vi "CreateMethodTree.vi"(6 "DisabledMethodsNames":T1(array[cluster]), 8 "error in (no error)":errorcluster, 9 "StartSelectedMethodsPerInterfaces":T1(array[cluster]), 10 "InterfacePath":T2[](array[typedef]), 11 "TreeControlRef":refnum<vi>) -> (0 "error out":errorcluster, 1 "InterfacesTag":string[](array[string]), 2 "MethodsTagPerInterfaces":cluster{"Array":string[]}[](array[cluster]), 3 "MethodsSelectedPerInterface":cluster{"Array":bool[]}[](array[cluster]), 4 "MethodsDisabledPerInterface":cluster{"Array":bool[]}[](array[cluster]))   [LabVIEW 2020, in "InterfaceLibrary.lvlib"]
uses:
  InterfaceLibrary.lvlib
  InterfaceInfo.ctl
  LvClass_class/GDSLvClass_ClassMethodInfo.ctl
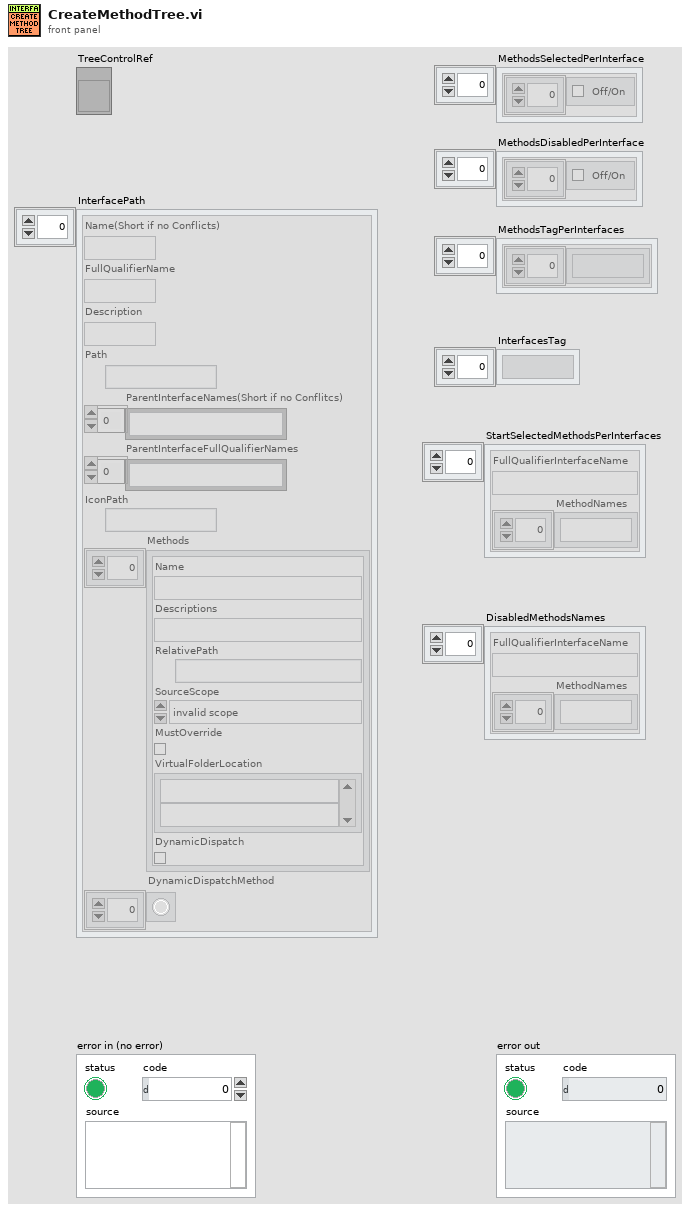
[diagram p1: front panel]
types:
  T1 = cluster{"FullQualifierInterfaceName":string, "MethodNames":string[]}[]
  T2 = typedef "InterfaceLibrary.lvlib/InterfaceInfo.ctl" = cluster{"Name(Short if no Conflicts)":string, "FullQualifierName":string, "Description":string, "Path":path, "ParentInterfaceNames(Short if no Conflitcs)":string[], "ParentInterfaceFullQualifierNames":string[], "IconPath":path, "Methods":T3[], "DynamicDispatchMethod":bool[]}
  T3 = typedef "GDSLvClass_ClassMethodInfo.ctl" = cluster{"Name":string, "Descriptions":string, "RelativePath":path, "SourceScope":enum32{"invalid scope", "public", "private", "protected", "community"}, "MustOverride":bool, "VirtualFolderLocation":string[], "DynamicDispatch":bool}
  T4 = cluster{"FullQualifierInterfaceName":string, "MethodNames":string[]}
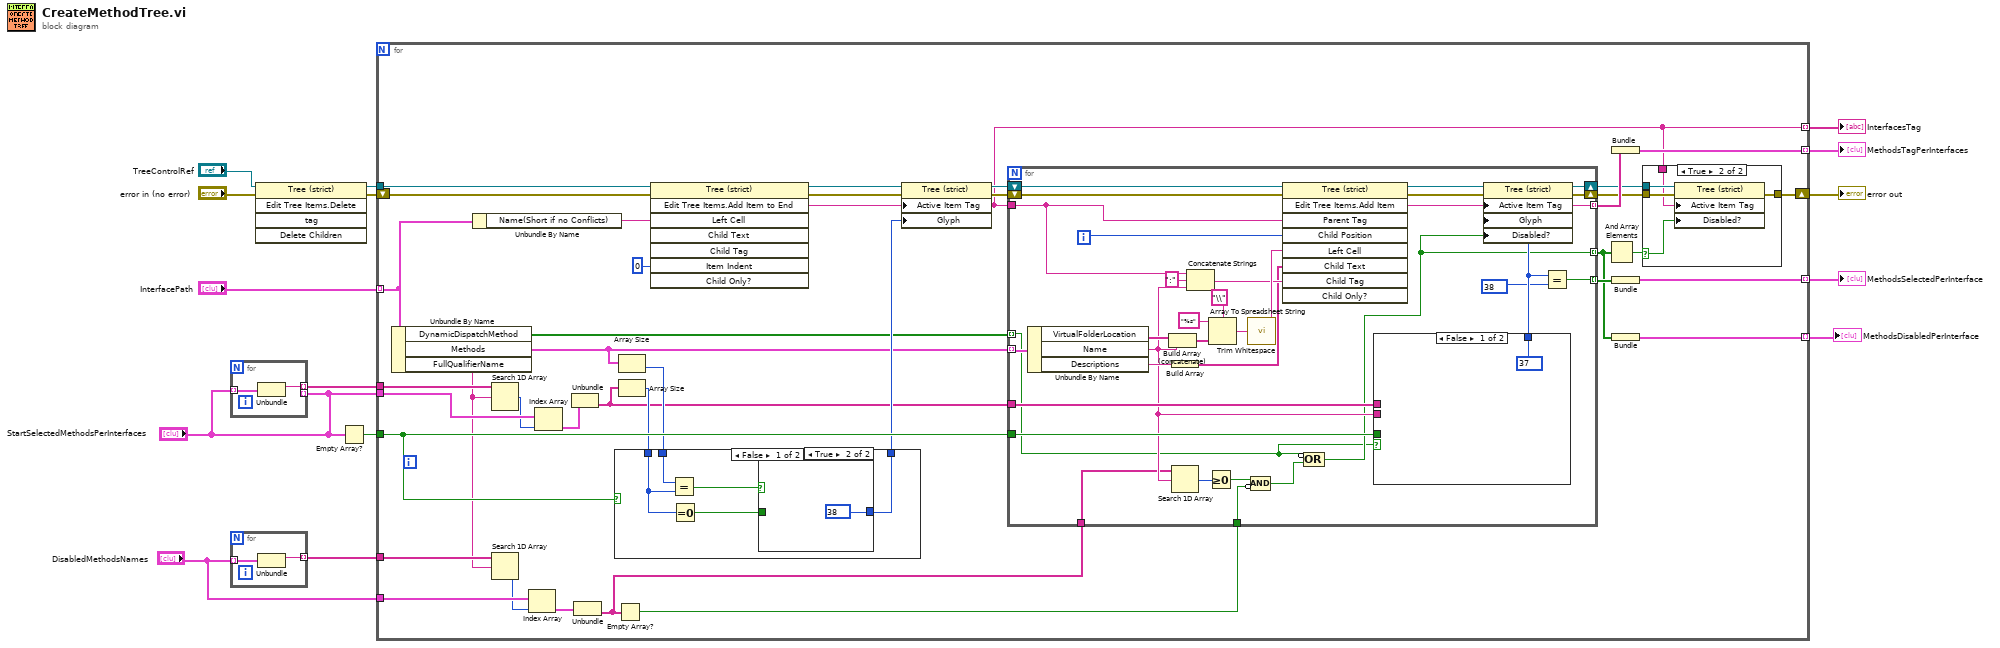
[diagram p0: block diagram]
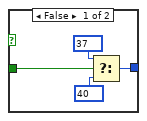
[diagram p3: hidden frame]
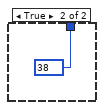
[diagram p4: hidden frame]
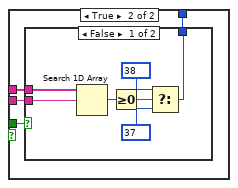
[diagram p5: hidden frame]
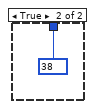
[diagram p6: hidden frame]
diagram:
  n1 = for {
    tunnel: "StartSelectedMethodsPerInterfaces" -> [w17] mode=indexing
    tunnel: [w16] -> w5 mode=indexing
    tunnel: "StartSelectedMethodsPerInterfaces" -> [_] mode=indexing
    n2 = Unbundle(w17) -> ("FullQualifierInterfaceName"=w16:string)  [unwired: 1 out]
  }
  n3 = for {
    tunnel: "DisabledMethodsNames" -> [w19] mode=indexing
    tunnel: [w18] -> w3 mode=indexing
    n4 = Unbundle(w19) -> ("FullQualifierInterfaceName"=w18:string)  [unwired: 1 out]
  }
  n5 = invoke on="Invoke Node" class="Tree (strict)" method="Edit Tree Items.Delete"(reference="TreeControlRef", error in="error in (no error)") -> (reference out=w14:refnum<vi>, error out=w7:errorcluster)  [unwired: 3 in, 3 out]
  n6 = Empty Array?(array="StartSelectedMethodsPerInterfaces") -> (empty?=w6:bool)
  n7 = for {
    tunnel: "InterfacePath" -> [w55] mode=indexing
    shift-right: [w25] -> w9
    shift-left: w7 -> [w52]
    tunnel: [w50] -> w11 mode=indexing
    tunnel: [w23] -> w10 mode=indexing
    tunnel: [w49] -> w12 mode=indexing
    tunnel: w14 -> [w48]
    tunnel: w6 -> [w45]
    tunnel: w5 -> [w40]
    tunnel: "StartSelectedMethodsPerInterfaces" -> [w39]
    tunnel: w3 -> [w35]
    tunnel: "DisabledMethodsNames" -> [w33]
    tunnel: [w21] -> w1 mode=indexing
    n8 = Unbundle By Name(w55) -> ("DynamicDispatchMethod"=w20:bool[], "Methods"=w43:T3[], "FullQualifierName"=w34:string)
    n9 = Unbundle By Name(w55) -> ("Name(Short if no Conflicts)"=w57:string)
    n10 = Search 1D Array(1D array=w40, element=w34) -> (index of element=w38:i32)  [unwired: 1 in]
    n11 = Search 1D Array(1D array=w35, element=w34) -> (index of element=w32:i32)  [unwired: 1 in]
    n12 = Index Array(array=w33, index=w32) -> (element=w31:T4)
    n13 = Index Array(array=w39, index=w38) -> (element=w37:T4)
    n14 = Unbundle(w37) -> ("MethodNames"=w36:string[])  [unwired: 1 out]
    n15 = Unbundle(w31) -> ("MethodNames"=w30:string[])  [unwired: 1 out]
    n16 = Empty Array?(array=w30) -> (empty?=w29:bool)
    n17 = Array Size(array=w43) -> (size(s)=w42:i32)
    n18 = Array Size(array=w36) -> (size(s)=w41:i32)
    n19 = case shown="False" w45 {
      tunnel: [w64 38] -> w44
      tunnel: w42 -> [w68 _]
      tunnel: w41 -> [w66 _]
      frame False {
        n20 = Equal?(x=w68, y=w66) -> (x = y?=w67:bool)
        n21 = Equal To 0?(x=w66) -> (x = 0?=w65:bool)
        n22 = case shown="True" w67 {
          tunnel: w65 -> [w70 _]
          tunnel: [w69 38] -> w64
          frame False {
            n23 = Select(t=37, s=w70, f=40) -> (s? t:f=w69:i32)
          }
          frame True {
          }
        }
      }
      frame True {
      }
    }
    n24 = invoke on="Invoke Node" class="Tree (strict)" method="Edit Tree Items.Add Item to End"(reference=w48, error in=w52, "Left Cell"=w57, "Item Indent"=0 ("New Item Indentation")) -> (reference out=w47:refnum<vi>, error out=w54:errorcluster, "Edit Tree Items:Add Item to End"=w23:string)  [unwired: 4 in, 5 out]
    n25 = property on="Property Node" class="Tree (strict)"(reference=w47, error in=w54, "Active Item Tag"=w23, "Glyph"=w44) -> (reference out=w46:refnum<vi>, error out=w53:errorcluster)
    n26 = for {
      tunnel: w43 -> [w107] mode=indexing
      tunnel: w23 -> [w96]
      shift-right: [w97] -> w26
      shift-left: w53 -> [w101]
      tunnel: [w87] -> w51 mode=indexing
      tunnel: w45 -> [w89]
      tunnel: w36 -> [w88]
      tunnel: w30 -> [w85]
      tunnel: w29 -> [w82]
      tunnel: [w79] -> w28 mode=indexing
      tunnel: [w76] -> w22 mode=indexing
      shift-right: [w78] -> w24
      shift-left: w46 -> [w91]
      tunnel: w20 -> [w75] mode=indexing
      i -> [w100]
      n27 = Unbundle By Name(w107) -> ("VirtualFolderLocation"=w106:string[], "Name"=w86:string, "Descriptions"=w93:string)
      n28 = Build Array (concatenate)(w106, w86) -> (w105:string[])
      n29 = Build Array(w93) -> (w92:string[])
      n30 = Search 1D Array(1D array=w85, element=w86) -> (index of element=w84:i32)  [unwired: 1 in]
      n31 = Concatenate Strings(w96, ":" ("string"), w86) -> (w95:string)
      n32 = Greater Or Equal To 0?(x=w84) -> (x >= 0?=w83:bool)
      n33 = Array To Spreadsheet String(delimiter (Tab)="\\", array=w105, 3:"%s" ("format string")) -> (spreadsheet string=w102:string)
      n34 = call <vilib>:"Trim Whitespace.vi"("string"=w102) -> ("trimmed string"=w99:string)  [unwired: 1 in]
      n35 = Compound Arithmetic op=AND(w83, invert w82) -> (w77:bool)
      n36 = invoke on="Invoke Node" class="Tree (strict)" method="Edit Tree Items.Add Item"(reference=w91, error in=w101, "Parent Tag"=w96, "Child Position"=w100, "Left Cell"=w99, "Child Text"=w92, "Child Tag"=w95) -> (reference out=w90:refnum<vi>, error out=w98:errorcluster, "Edit Tree Items:Add Item"=w87:string)  [unwired: 2 in, 6 out]
      n37 = Compound Arithmetic op=OR(invert w75, w77) -> (w76:bool)
      n38 = case shown="False" w75 {
        tunnel: w89 -> [_ w112]
        tunnel: w88 -> [_ w111]
        tunnel: w86 -> [_ w110]
        tunnel: [37 w109] -> w81
        frame False {
        }
        frame True {
          n39 = case shown="False" w112 {
            tunnel: [w113 38] -> w109
            tunnel: w111 -> [w119 _]
            tunnel: w110 -> [w118 _]
            frame False {
              n40 = Search 1D Array(1D array=w119, element=w118) -> (index of element=w117:i32)  [unwired: 1 in]
              n41 = Greater Or Equal To 0?(x=w117) -> (x >= 0?=w116:bool)
              n42 = Select(t=38, s=w116, f=37) -> (s? t:f=w113:i32)
            }
            frame True {
            }
          }
        }
      }
      n43 = property on="Property Node" class="Tree (strict)"(reference=w90, error in=w98, "Active Item Tag"=w87, "Glyph"=w81, "Disabled?"=w76) -> (reference out=w78:refnum<vi>, error out=w97:errorcluster)
      n44 = Equal?(x=w81, y=38) -> (x = y?=w79:bool)
    }
    n45 = And Array Elements(Boolean array=w22) -> (logical AND=w27:bool)
    n46 = Bundle(w51) -> (w50:cluster{string[]})  [unwired: 1 in]
    n47 = Bundle(w28) -> (w49:cluster{bool[]})  [unwired: 1 in]
    n48 = Bundle(w22) -> (w21:cluster{bool[]})  [unwired: 1 in]
    n49 = case shown="True" w27 {
      selector: w27 -> [_ w59]
      tunnel: w26 -> [w58 w63]
      tunnel: [w58 w62] -> w25
      tunnel: w24 -> [_ w61]
      tunnel: w23 -> [_ w60]
      frame False {
      }
      frame True {
        n50 = property on="Property Node" class="Tree (strict)"(reference=w61, error in=w63, "Active Item Tag"=w60, "Disabled?"=w59) -> (error out=w62:errorcluster)  [unwired: 1 out]
      }
    }
  }
  "MethodsSelectedPerInterface" <- w12
  "MethodsTagPerInterfaces" <- w11
  "InterfacesTag" <- w10
  "error out" <- w9
  "MethodsDisabledPerInterface" <- w1
